vi "Own20261012_ConnectSourceToStructure.vi"() -> ()   [LabVIEW 2024]
panel:
  out "error out":errorcluster caption="错误输出"
  in  "source_terminal":u32
  in  "structure_id":u32
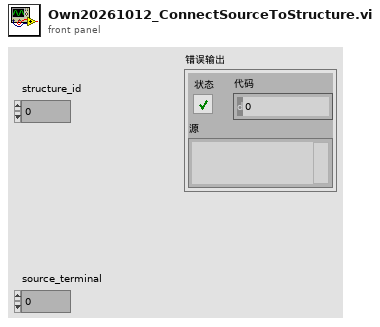
[diagram p1: front panel]
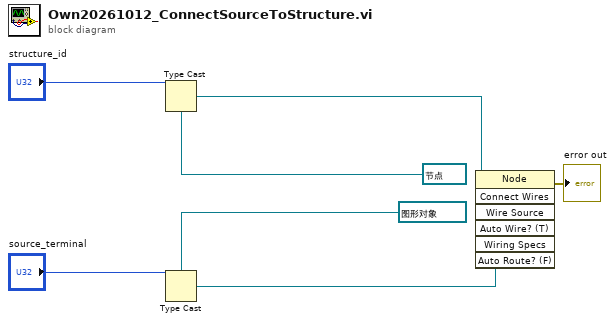
[diagram p0: block diagram]
diagram:
  n1 = Type Cast(type=refnum<vi> refnum ("引用"), x="structure_id") -> (*(type *) &x=w5:refnum<vi>)
  n2 = Type Cast(type=refnum<vi> refnum ("连线源"), x="source_terminal") -> (*(type *) &x=w2:refnum<vi>)
  n3 = invoke class="Node" method="Connect Wires"(reference=w5, "Wire Source"=w2) -> (error out=→"error out":errorcluster)  [unwired: 5 in, 6 out]
